vi "Handle Processing Error.vi"(8 "error in (no error)":errorcluster, 11 "Nominal-Streamer in":refnum<class "Nominal-Streamer.lvclass">) -> (0 "error out":errorcluster, 2 "Error Response":T1, 3 "Nominal-Streamer out":refnum<class "Nominal-Streamer.lvclass">)   [LabVIEW 2020, in "Nominal-Streamer.lvlib" / "Nominal-Streamer.lvclass"]
uses:
  Nominal-Streamer.lvclass
  <vilib>/FlexLogger/SDK/PluginSDK.lvlibp/PEFClasses/SDK/Processing Element/Error Response Type.ctl
  <vilib>/FlexLogger/SDK/PluginSDK.lvlibp/PEFClasses/SDK/Processing Element/Processing Element.lvclass
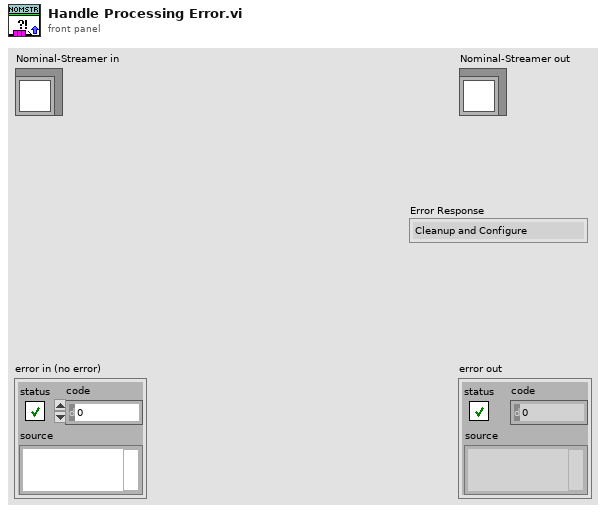
[diagram p1: front panel]
types:
  T1 = typedef "PluginSDK.lvlibp/Processing Element.lvclass/Error Response Type.ctl" = enum16{"Cleanup and Configure", "Cleanup and Finalize", "Report and Continue"}
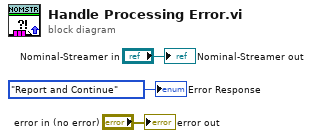
[diagram p0: block diagram]
diagram:
  "error out" <- "error in (no error)"
  "Nominal-Streamer out" <- "Nominal-Streamer in"
  "Error Response" <- Error_Response_Type."Report and Continue" ("Error Response")
